vi "W11_Alarm_TempLow_test.vi"() -> ()   [LabVIEW 2018]
doc: "Use this template to build a VI to use as a subVI."
panel:
  out "lamp[]":bool[](array[boolean])
  out "alarm[]":bool[](array[boolean])
  out "below[]":bool[](array[boolean])
  in  "setpoint C":dbl
  in  "ack[]":bool[](array[boolean])
  in  "temperature[]":dbl[](array[numeric])
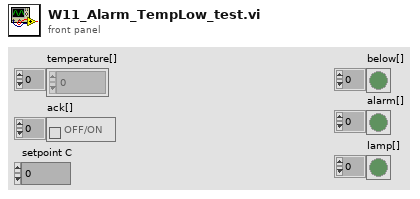
[diagram p1: front panel]
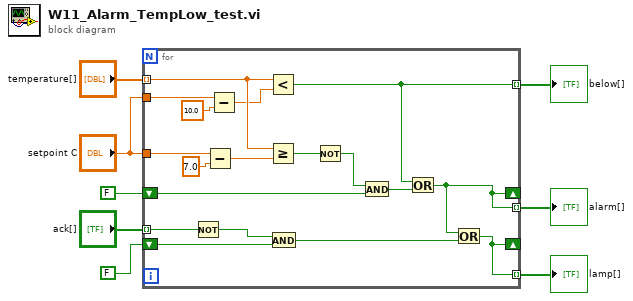
[diagram p0: block diagram]
diagram:
  n1 = for {
    shift-right: [w10] -> _
    shift-left: FALSE -> [w17]
    shift-right: [w9] -> _
    shift-left: FALSE -> [w13]
    tunnel: "temperature[]" -> [w24] mode=indexing
    tunnel: "ack[]" -> [w15] mode=indexing
    tunnel: "setpoint C" -> [w26]
    tunnel: "setpoint C" -> [w22]
    tunnel: [w11] -> w3 mode=indexing
    tunnel: [w10] -> w2 mode=indexing
    tunnel: [w9] -> w1 mode=indexing
    n2 = Not(x=w15) -> (.not. x?=w14:bool)
    n3 = Subtract(x=w22, y=7.0) -> (x-y=w20:dbl)
    n4 = Subtract(x=w26, y=10.0) -> (x-y=w23:dbl)
    n5 = Less?(x=w24, y=w23) -> (x < y?=w11:bool)
    n6 = Greater Or Equal?(x=w24, y=w20) -> (x >= y?=w19:bool)
    n7 = And(x=w14, y=w13) -> (x .and. y?=w12:bool)
    n8 = Not(x=w19) -> (.not. x?=w18:bool)
    n9 = And(x=w18, y=w17) -> (x .and. y?=w16:bool)
    n10 = Or(x=w11, y=w16) -> (x .or. y?=w10:bool)
    n11 = Or(x=w10, y=w12) -> (x .or. y?=w9:bool)
  }
  "below[]" <- w3
  "alarm[]" <- w2
  "lamp[]" <- w1
